vi "VirtualATE_V3.vi"() -> ()   [LabVIEW 2026]
uses:
  <vilib>/NI/Modbus Library/API/Modbus API.lvclass/Modbus API.ctl
  <vilib>/NI/Modbus Library/Transmission Data Unit/Transmission Data Unit.lvclass/Transmission Data Unit.ctl
  <vilib>/NI/Modbus Library/Transmission Data Unit/Write Unit ID.vi
  <vilib>/NI/Modbus Library/API/Read Transmission Data Unit.vi
  <vilib>/NI/Modbus Library/API/Write Transmission Data Unit.vi
  <vilib>/NI/Modbus Library/API/Master/Modbus Master.lvclass
  <vilib>/NI/Modbus Library/API/Wrapper/Create TCP Master.vi
  <vilib>/NI/Modbus Library/API/Wrapper/API Main.lvlib
panel:
  in  "Tab Control":enum32{"검사 운영", "통신 진단"}(tab)
  in  "AutoVoltage":bool=TRUE
  in  "SimVoltage_mV":i32=3300
  in  "Low_mV":i32=3000
  in  "High_mV":i32=3600
  in  "검사 결과 선택":enum16{"PASS", "FAIL", "RETEST"}(ring)
  out "ACTIVE_ID":u16
  out "ACTIVE_RESULT":u16
  out "ACTIVE_RECORD":string
  in  "Server IP":string="192.168.0.5"
  in  "Port":u16=1502
  in  "Unit ID":u8=1
  out "error out":errorcluster
  out "처리 메시지":string
  in  "LogFilePath":path
  out "ATE_STATE":u16
  out "ATE_READY":bool
  out "PLC_LIVE_OK":bool
  in  "ATE 읽기 정지":bool
  out "ATE_REQUEST":u16
  out "ATE_REQUEST_ID":u16
  out "ATE_RESULT":u16
  out "ATE_RESPONSE_ID":u16
  out "ATE_DONE":u16
  out "TEEST_RESULT_LATCH":u16
  out "SEQ_STATE":u16
  out "ALARM_CODE":u16
  out "PLC_RX_RESULT":u16
  out "PLC_RX_DONE":u16
  out "PLC_RX_RESPONSE_ID":u16
  out "PLC_ACCEPTED_ID":u16
  out "PLC_LIVE_COUNTER":u16
  out "수신 레지스터":u16[](array[numeric])
  out "마지막 Modbus 읽기 정상":bool
  out "PLC_HB_TIMEOUT":bool
  out "STATE_ELAPSED_MS":u32
  out "PLC_HB_AGE_MS":u32
  out "바깥 Tick Count(ms)":u32
  # "검사 조건"
  # "진행 중 검사"
  # "활성 요청 ID"
  # "전압 기준 자동 판정"
  # "가상 전압(mV)"
  # "하한(mV)"
  # "상한(mV)"
  # "활성 결과코드"
  # "0 없음    1 PASS    2 FAIL    3 RETEST"
  # "자동 판정 OFF 일 때 사용"
  # "캡처한 검사 레코드"
  # "Modbus 접속 설정 (실행 전)"
  # "서버 IP"
  # "포트"
  # "국번"
  # "수신 레지스터"
  # "R[1]"
  # "검사 요청"
  # "R[8]"
  # "LS 알람 코드"
  # "R[2]"
  # "검사 요청 ID"
  # "R[9]"
  # "PLC 수신 결과"
  # "R[3]"
  # "ATE 결과 워드"
  # "PLC 수신 DONE"
  # "R[10]"
  # "R[4]"
  # "ATE 응답 ID"
  # "R[11]"
  # "PLC 수신 응답 ID"
  # "R[5]"
  # "ATE 완료 워드"
  # "R[12]"
  # "PLC 수락 ID"
  # "R[6]"
  # "PLC 수락 결과"
  # "PLC 생존 카운터"
  # "R[13]"
  # "R[7]"
  # "LS 공정 상태"
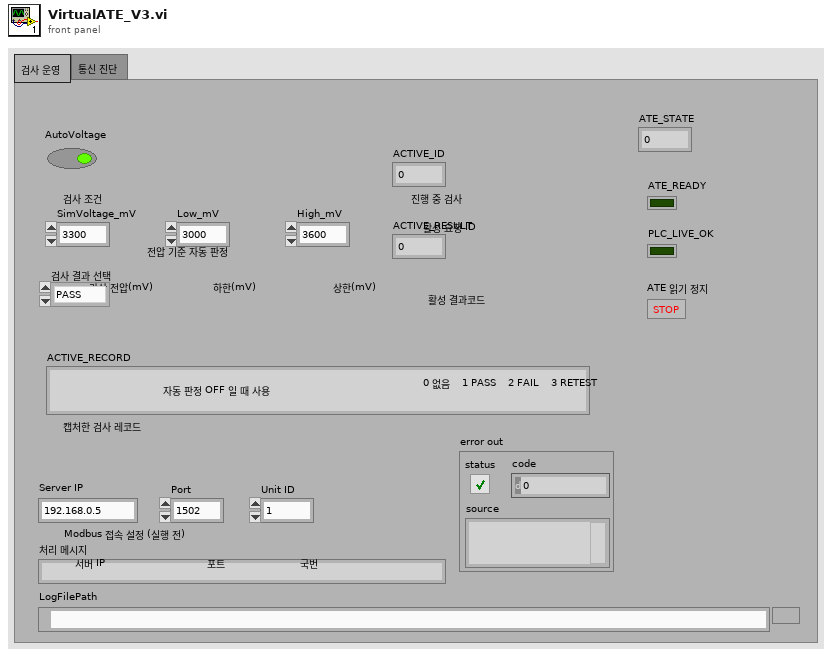
[diagram p1: front panel]
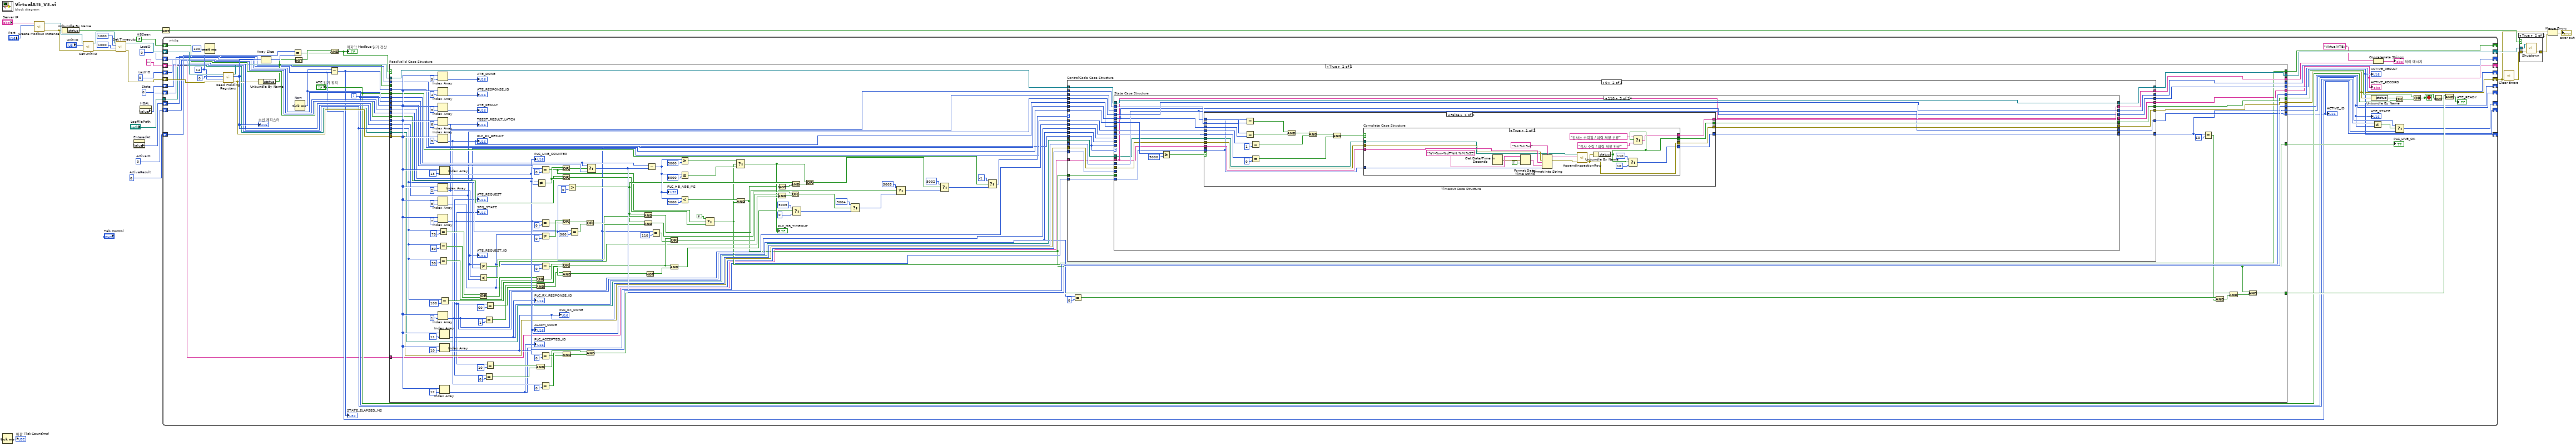
[diagram p0: block diagram]
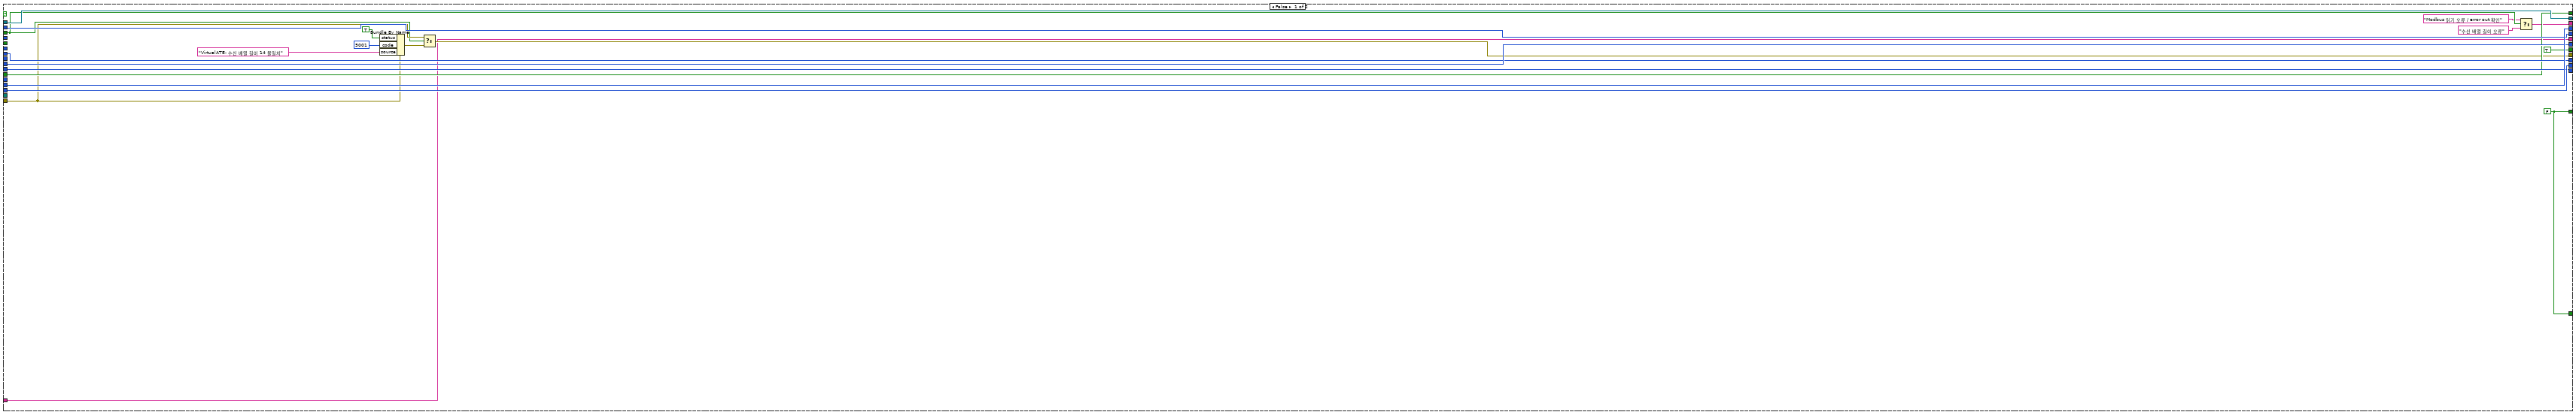
[diagram p3: hidden frame]
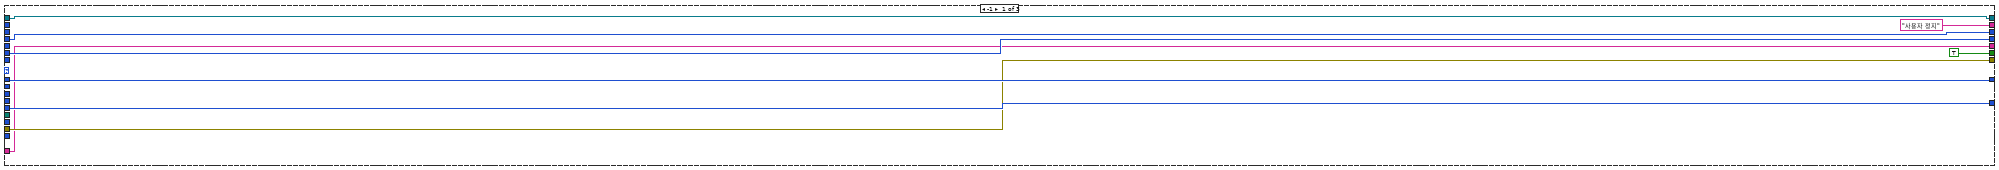
[diagram p4: hidden frame]
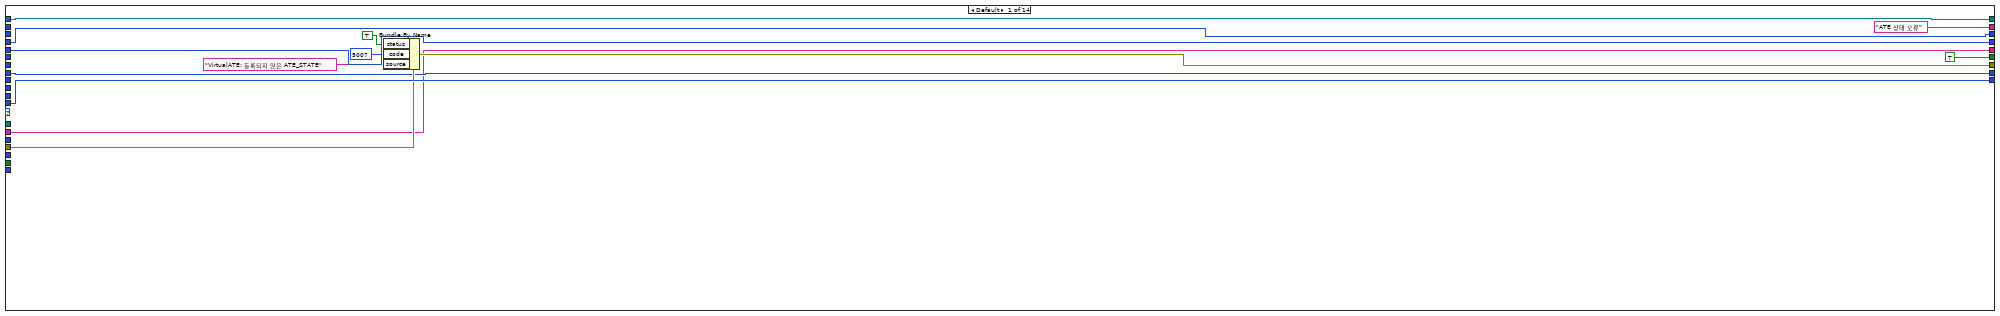
[diagram p5: hidden frame]
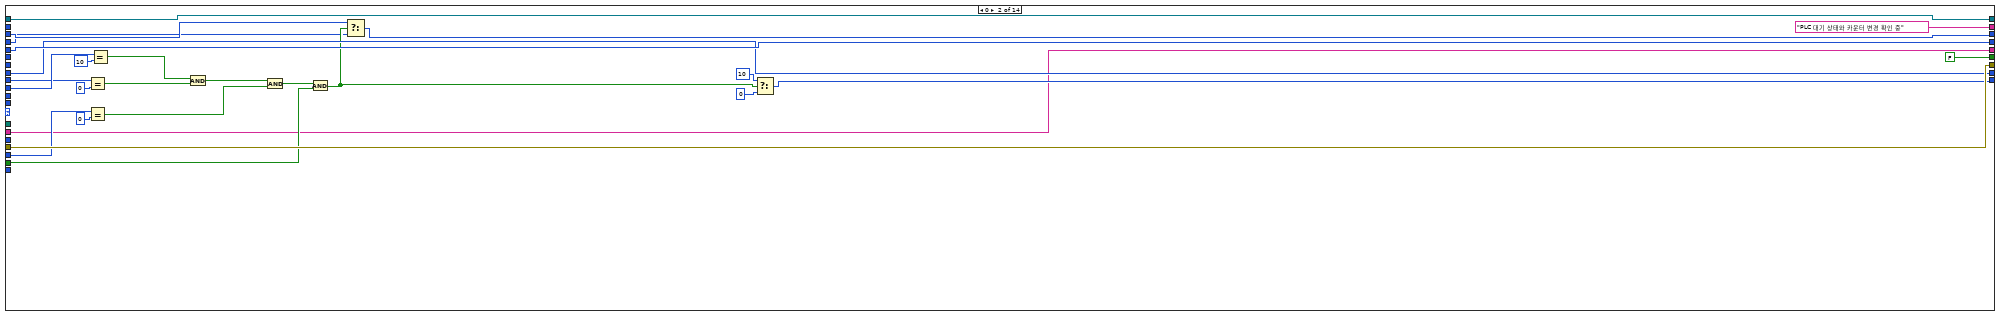
[diagram p6: hidden frame]
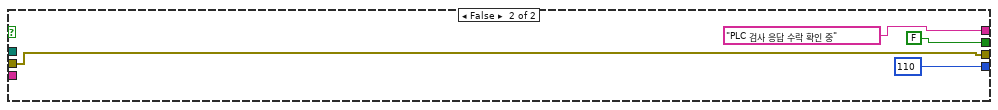
[diagram p7: hidden frame]
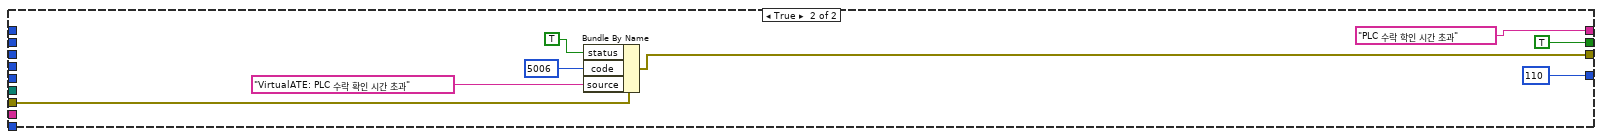
[diagram p8: hidden frame]
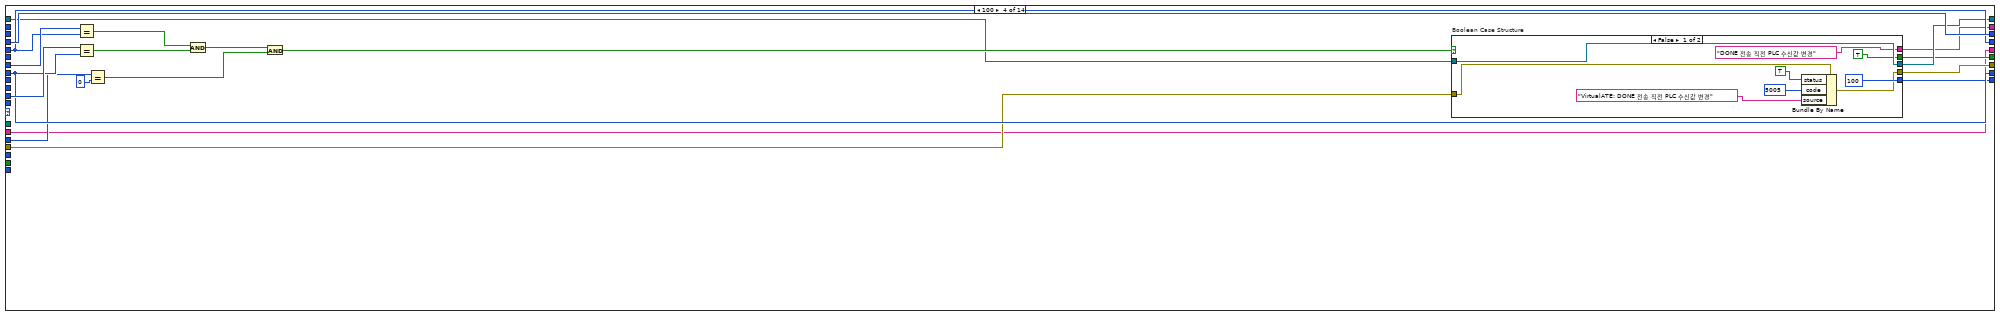
[diagram p9: hidden frame]
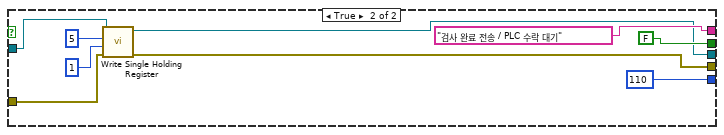
[diagram p10: hidden frame]
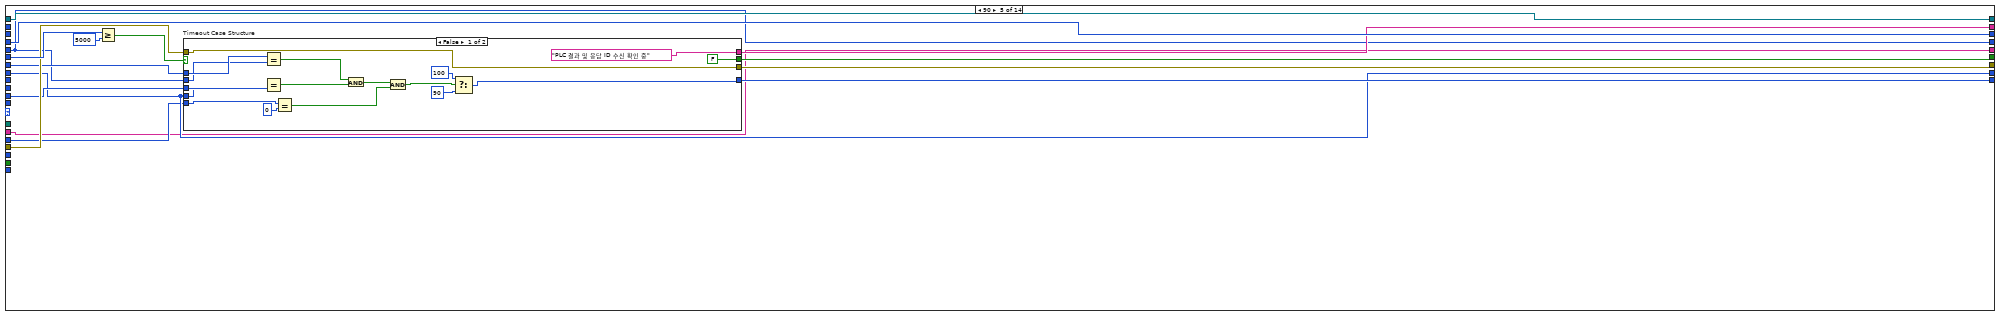
[diagram p11: hidden frame]
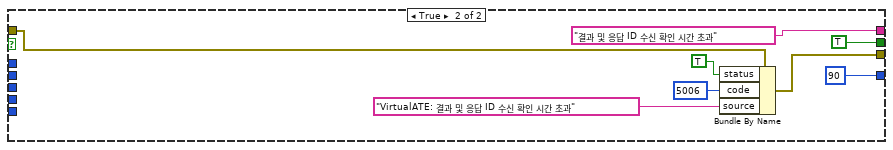
[diagram p12: hidden frame]
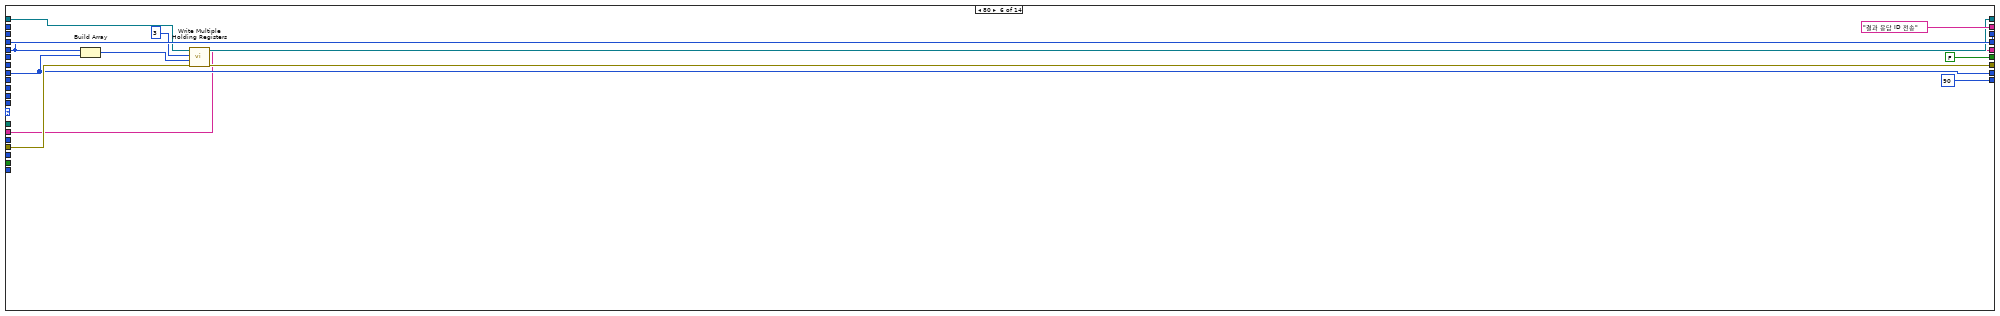
[diagram p13: hidden frame]
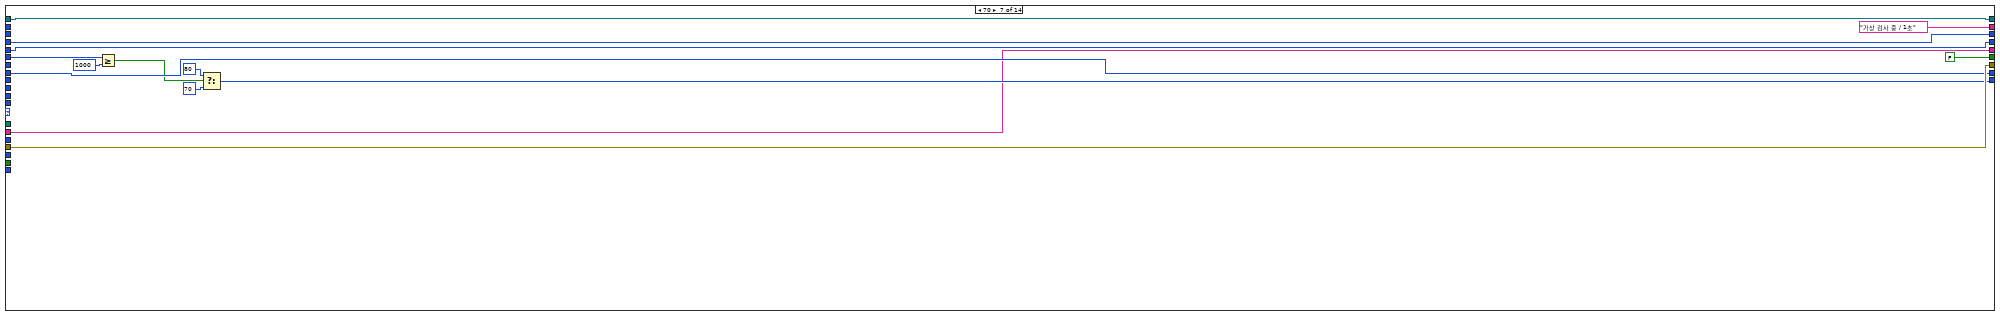
[diagram p14: hidden frame]
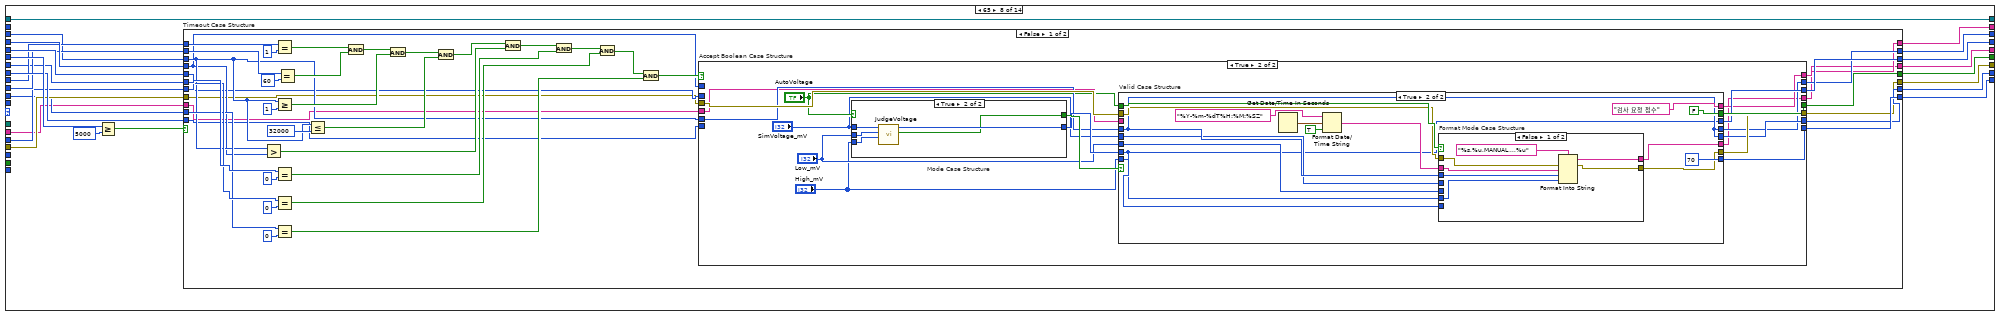
[diagram p15: hidden frame]
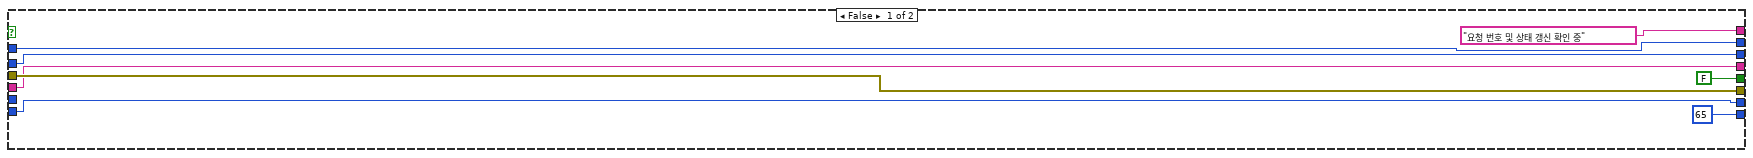
[diagram p16: hidden frame]
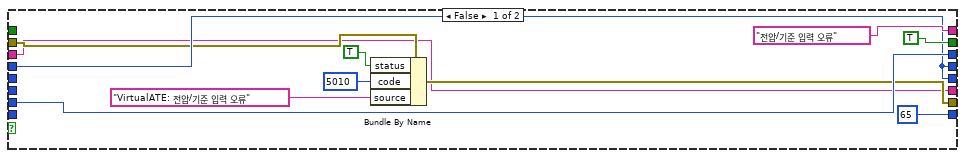
[diagram p17: hidden frame]
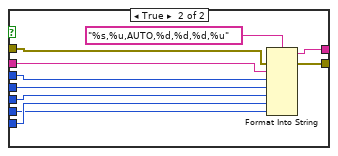
[diagram p18: hidden frame]
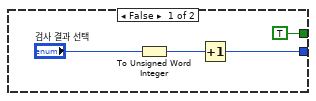
[diagram p19: hidden frame]
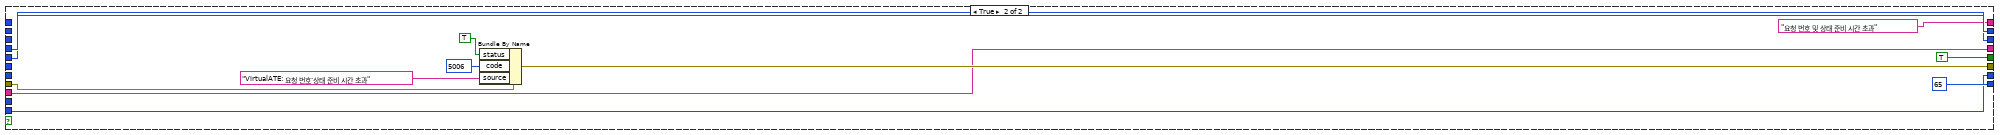
[diagram p20: hidden frame]
diagram:
  w11 = FALSE  # HBSeen
  w6 = u16 0  # LastHB
  w7 = u16 0  # ActiveResult
  w8 = u16 0  # ActiveID
  w9 = u16 0  # LastID
  w10 = u16 0  # State
  n1 = Tick Count (ms)() -> (millisecond timer value=→"바깥 Tick Count(ms)":u32)
  n2 = call-poly <vilib>:"Create Modbus Instance.vi"("port (502)"="Port", "address"="Server IP") -> ("error out"=w19:errorcluster, "TCP master instance"=w24:refnum<class "Modbus Master.lvclass">)  [unwired: 8 in]
  n3 = Unbundle By Name(w19) -> ("status"=w18:bool)
  n4 = call <vilib>:"Set Unit ID.vi"("error in"=w19, "unit ID"="Unit ID", "Modbus master in"=w24) -> ("error out"=w22:errorcluster, "Modbus master out"=w23:refnum<class "Modbus Master.lvclass">)  [unwired: 7 in]
  n5 = call <vilib>:"Set Timeouts.vi"("error in"=w22, "write operation timeout"=1000, "read operation timeout"=1000, "Modbus master in"=w23) -> ("error out"=w20:errorcluster, "Modbus master out"=w21:refnum<class "Modbus Master.lvclass">)  [unwired: 6 in]
  n6 = property on="EnteredAt" class="DigNum (strict)"() -> ("Value"=w4:u32)  [unwired: 2 in, 2 out]
  n7 = property on="HBAt" class="DigNum (strict)"() -> ("Value"=w3:u32)  [unwired: 2 in, 2 out]
  n8 = Not(x=w18) -> (.not. x?=w17:bool)
  n9 = while {
    shift-right: [w53] -> w13
    shift-left: w20 -> [w76]
    shift-right: [w64] -> w16
    shift-left: w21 -> [w77]
    shift-right: [w33] -> _
    shift-left: w10 -> [w45]
    shift-right: [w68] -> _
    shift-left: w9 -> [w69]
    shift-right: [w35] -> _
    shift-left: w8 -> [w67]
    shift-right: [w34] -> _
    shift-left: w7 -> [w66]
    shift-right: [w43] -> _
    shift-left: w3 -> [w60]
    shift-right: [w61] -> _
    shift-left: w6 -> [w62]
    shift-right: [w47] -> _
    shift-left: w4 -> [w44]
    shift-right: [w42] -> _
    shift-left: w11 -> [w59]
    shift-right: [w31] -> _
    shift-left: "" -> [w32]
    tunnel: "LogFilePath" -> [w30]
    i -> [w48]
    stop <- w50 stop-if-true
    w75 = u16 14 ("number of inputs")
    n10 = Wait (ms)(milliseconds to wait=u32 100) -> ()  [unwired: 1 out]
    n11 = call-dynamic "Read Holding Registers.vi"("error in"=w76, "number of inputs"=w75, "starting address"=u16 0, "Modbus master in"=w77) -> ("error out"=w63:errorcluster, "register values"=w71:u16[], "Modbus master out"=w65:refnum<class "Modbus Master.lvclass">)  [unwired: 5 in]
    "수신 레지스터" <- w71
    n12 = Unbundle By Name(w63) -> ("status"=w58:bool)
    n13 = Array Size(array=w71) -> (size(s)=w74:i32)
    n14 = Equal?(x=w75, y=w74) -> (x = y?=w72:bool)
    n15 = Not(x=w58) -> (.not. x?=w73:bool)
    n16 = Tick Count (ms) "Now"() -> (millisecond timer value=w41:u32)
    n17 = And(x=w73, y=w72) -> (x .and. y?=w70:bool)
    "마지막 Modbus 읽기 정상" <- w70
    n18 = Subtract(x=w41, y=w44) -> (x-y=w39:u32)
    "STATE_ELAPSED_MS" <- w39
    n19 = case "ReadValid Case Structure" shown="True" w70 {
      tunnel: w71 -> [_ w229]
      tunnel: w45 -> [w100 w136]
      tunnel: [w100 w130] -> w33
      tunnel: w69 -> [w99 w148]
      tunnel: [w99 w147] -> w68
      tunnel: w67 -> [w98 w146]
      tunnel: [w98 w145] -> w35
      tunnel: w66 -> [w97 w144]
      tunnel: [w97 w143] -> w34
      tunnel: w65 -> [w96 w142]
      tunnel: [w96 w141] -> w64
      tunnel: w63 -> [w88 w140]
      tunnel: [w82 w139] -> w53
      tunnel: w62 -> [w95 w221]
      tunnel: [w95 w218] -> w61
      tunnel: w60 -> [w94 w216]
      tunnel: [w94 w217] -> w43
      tunnel: w59 -> [w93 w219]
      tunnel: [w93 w111] -> w42
      tunnel: w58 -> [w86 _]
      tunnel: [TRUE w137] -> w56
      tunnel: [w83 w138] -> w37
      tunnel: [w81 w117] -> w54
      tunnel: [w81 w104] -> w49
      tunnel: w48 -> [_ w223]
      tunnel: w41 -> [_ w210]
      tunnel: "ATE 읽기 정지" -> [_ w150]
      tunnel: w39 -> [_ w116]
      tunnel: w32 -> [w80 w103]
      tunnel: [w80 w102] -> w31
      tunnel: w30 -> [_ w101]
      frame False {
        w81 = FALSE
        n20 = Bundle By Name(cluster=w88, "status"=TRUE, "code"=5001, "source"="VirtualATE: 수신 배열 길이 14 불일치") -> (w89:errorcluster)
        n21 = Select(t=w88, s=w86, f=w89) -> (s? t:f=w82:errorcluster)
        n22 = Select(t="Modbus 읽기 오류 / error out 확인", s=w86, f="수신 배열 길이 오류") -> (s? t:f=w83:string)
      }
      frame True {
        n23 = Index Array(array=w229, index=5) -> (element=→"ATE_DONE":u16)
        n24 = Index Array(array=w229, index=4) -> (element=→"ATE_RESPONSE_ID":u16)
        n25 = Index Array(array=w229, index=3) -> (element=→"ATE_RESULT":u16)
        n26 = Index Array(array=w229, index=6) -> (element=w105:u16)
        "TEEST_RESULT_LATCH" <- w105
        n27 = Index Array(array=w229, index=9) -> (element=w114:u16)
        "PLC_RX_RESULT" <- w114
        n28 = Index Array(array=w229, index=2) -> (element=w107:u16)
        "ATE_REQUEST_ID" <- w107
        n29 = Index Array(array=w229, index=8) -> (element=w108:u16)
        "ALARM_CODE" <- w108
        n30 = Index Array(array=w229, index=7) -> (element=w109:u16)
        "SEQ_STATE" <- w109
        n31 = Index Array(array=w229, index=1) -> (element=w112:u16)
        "ATE_REQUEST" <- w112
        n32 = Equal?(x=w136, y=u16 70) -> (x = y?=w199:bool)
        n33 = Equal?(x=w136, y=u16 80) -> (x = y?=w198:bool)
        n34 = Equal?(x=w136, y=u16 90) -> (x = y?=w197:bool)
        n35 = Index Array(array=w229, index=13) -> (element=w218:u16)
        "PLC_LIVE_COUNTER" <- w218
        n36 = Index Array(array=w229, index=11) -> (element=w113:u16)
        "PLC_RX_RESPONSE_ID" <- w113
        n37 = Index Array(array=w229, index=10) -> (element=w115:u16)
        "PLC_RX_DONE" <- w115
        n38 = Index Array(array=w229, index=12) -> (element=w106:u16)
        "PLC_ACCEPTED_ID" <- w106
        n39 = Equal?(x=w136, y=u16 100) -> (x = y?=w195:bool)
        n40 = Not Equal?(x=w107, y=w146) -> (x != y?=w179:bool)
        n41 = Less?(x=w107, y=w148) -> (x < y?=w181:bool)
        n42 = Or(x=w199, y=w198) -> (x .or. y?=w196:bool)
        n43 = Equal?(x=w112, y=u16 1) -> (x = y?=w188:bool)
        n44 = Equal?(x=w112, y=u16 0) -> (x = y?=w127:bool)
        n45 = Equal?(x=w109, y=u16 60) -> (x = y?=w187:bool)
        n46 = Equal?(x=w109, y=u16 10) -> (x = y?=w128:bool)
        n47 = Or(x=w196, y=w197) -> (x .or. y?=w194:bool)
        n48 = And(x=w188, y=w187) -> (x .and. y?=w185:bool)
        n49 = And(x=w128, y=w127) -> (x .and. y?=w122:bool)
        n50 = Not Equal?(x=w218, y=w221) -> (x != y?=w220:bool)
        n51 = Equal?(x=w223, y=0) -> (x = y?=w110:bool)
        n52 = Equal?(x=w109, y=u16 0) -> (x = y?=w172:bool)
        n53 = Not Equal?(x=w108, y=u16 0) -> (x != y?=w173:bool)
        n54 = Equal?(x=w108, y=u16 0) -> (x = y?=w186:bool)
        n55 = Equal?(x=w115, y=u16 0) -> (x = y?=w125:bool)
        n56 = Equal?(x=w114, y=u16 0) -> (x = y?=w126:bool)
        n57 = Or(x=w220, y=w110) -> (x .or. y?=w214:bool)
        n58 = Or(x=w219, y=w220) -> (x .or. y?=w215:bool)
        n59 = Or(x=w173, y=w172) -> (x .or. y?=w171:bool)
        n60 = Or(x=w194, y=w195) -> (x .or. y?=w182:bool)
        n61 = And(x=w185, y=w186) -> (x .and. y?=w184:bool)
        n62 = And(x=w126, y=w125) -> (x .and. y?=w121:bool)
        n63 = Greater?(x=w136, y=u16 0) -> (0:w168:bool)
        n64 = Equal?(x=w109, y=u16 900) -> (x = y?=w170:bool)
        n65 = Or(x=w171, y=w170) -> (x .or. y?=w169:bool)
        n66 = And(x=w122, y=w121) -> (x .and. y?=w119:bool)
        n67 = Select(t=w210, s=w214, f=w216) -> (s? t:f=w217:u32)
        n68 = And(x=w168, y=w169) -> (x .and. y?=w160:bool)
        n69 = And(x=w168, y=w181) -> (x .and. y?=w178:bool)
        n70 = Not(x=w184) -> (.not. x?=w183:bool)
        n71 = Subtract(x=w210, y=w217) -> (x-y=w209:u32)
        "PLC_HB_AGE_MS" <- w209
        n72 = Equal?(x=w136, y=u16 110) -> (x = y?=w192:bool)
        n73 = Or(x=w182, y=w192) -> (x .or. y?=w180:bool)
        n74 = And(x=w182, y=w183) -> (x .and. y?=w164:bool)
        n75 = Greater Or Equal?(x=w209, y=u32 3000) -> (x >= y?=w206:bool)
        n76 = Greater Or Equal?(x=w209, y=u32 5000) -> (x >= y?=w205:bool)
        n77 = Less?(x=w209, y=u32 3000) -> (x < y?=w212:bool)
        n78 = Select(t=FALSE, s=w110, f=w215) -> (s? t:f=w111:bool)
        n79 = Select(t=w206, s=w111, f=w205) -> (s? t:f=w165:bool)
        "PLC_HB_TIMEOUT" <- w165
        n80 = And(x=w212, y=w111) -> (x .and. y?=w104:bool)
        n81 = Not(x=w104) -> (.not. x?=w167:bool)
        n82 = And(x=w180, y=w179) -> (x .and. y?=w177:bool)
        n83 = Or(x=w178, y=w177) -> (x .or. y?=w161:bool)
        n84 = And(x=w168, y=w167) -> (x .and. y?=w166:bool)
        n85 = Select(t=5005, s=w164, f=0) -> (s? t:f=w157:i32)
        n86 = Or(x=w165, y=w166) -> (x .or. y?=w159:bool)
        n87 = Select(t=5004, s=w161, f=w157) -> (s? t:f=w156:i32)
        n88 = Select(t=5003, s=w160, f=w156) -> (s? t:f=w154:i32)
        n89 = Select(t=5002, s=w159, f=w154) -> (s? t:f=w152:i32)
        n90 = Select(t=-1, s=w150, f=w152) -> (s? t:f=w149:i32)
        n91 = case "ControlCode Case Structure" shown="0" w149 {
          selector: w149 -> [_ _ w817]
          tunnel: w136 -> [w249 w260 w825]
          tunnel: [w249 w271 w825] -> w130
          tunnel: w148 -> [w248 w277 w824]
          tunnel: [w248 w268 w824] -> w147
          tunnel: w146 -> [w247 w276 w823]
          tunnel: [w247 w267 w823] -> w145
          tunnel: [w246 w273 w822] -> w143
          tunnel: w144 -> [w246 w275 w822]
          tunnel: [w245 w272 w821] -> w141
          tunnel: w142 -> [w245 w274 w821]
          tunnel: [w244 w270 w820] -> w139
          tunnel: w140 -> [w244 w269 w819]
          tunnel: ["사용자 정지" w265 w799] -> w138
          tunnel: [TRUE w266 TRUE] -> w137
          tunnel: w116 -> [_ w264 _]
          tunnel: w115 -> [_ w263 _]
          tunnel: w114 -> [_ w262 _]
          tunnel: w113 -> [_ w261 _]
          tunnel: w112 -> [_ w257 _]
          tunnel: w109 -> [_ w259 _]
          tunnel: w108 -> [_ w258 _]
          tunnel: w107 -> [_ w256 _]
          tunnel: w106 -> [_ w255 _]
          tunnel: w105 -> [_ w254 _]
          tunnel: w104 -> [_ w253 _]
          tunnel: w103 -> [w241 w252 w798]
          tunnel: [w241 w251 w798] -> w102
          tunnel: w101 -> [_ w250 _]
          frame -1 {
          }
          frame 0 {
            n92 = case "State Case Structure" shown="110" w260 {
              tunnel: w277 -> [w279 w293 w333 w407 w440 w478 w490 w511 w658 w692 w710 w751 w765 w795]
              tunnel: w276 -> [w280 w313 w320 w403 w428 w468 w489 w507 w657 w691 w709 w750 w764 w794]
              tunnel: w275 -> [w289 w316 w319 w405 w430 w469 w493 w505 w661 w695 w712 w753 w767 w797]
              tunnel: w274 -> [w288 w315 w334 w393 w441 w472 w492 w516 w660 w694 w711 w747 w766 w791]
              tunnel: [w289 w316 w319 w405 w430 w469 w493 w504 w661 w695 w712 w753 w767 w797] -> w273
              tunnel: [w288 w315 w334 w392 w441 w470 w492 w516 w660 w694 w711 w745 w766 w790] -> w272
              tunnel: [w290 w295 w329 w390 w434 u16 90 w484 w512 w649 w665 w703 u16 40 w758 u16 20] -> w271
              tunnel: [w283 w314 w325 w394 w435 w471 w491 w502 w659 w693 w701 w744 w757 w789] -> w270
              tunnel: w269 -> [w287 w314 w326 w395 w436 w473 w491 w503 w659 w693 w702 w746 w756 w788]
              tunnel: [w279 w292 w333 w407 w440 w478 w490 w510 w658 w692 w710 w751 w765 w795] -> w268
              tunnel: [w280 w313 w320 w403 w428 w468 w489 w506 w657 w691 w709 w750 w764 w794] -> w267
              tunnel: [TRUE FALSE w328 w391 w433 FALSE FALSE w509 FALSE FALSE w705 FALSE w759 FALSE] -> w266
              tunnel: ["ATE 상태 오류" "PLC 대기 상태와 카운터 변경 확인 중" w327 w389 w432 "결과 응답 ID 전송" "가상 검사 중 / 1초" w508 "새 검사 요청 대기" "분류 및 배출 완료 후 PLC 대기 복귀 확인" w704 "결과 및 응답 ID 초기화 전송" w760 "DONE=0 전송 / PLC 반영 대기"] -> w265
              tunnel: w260 -> [w290 _ _ _ _ _ _ _ _ _ _ _ _ _]
              tunnel: w264 -> [_ _ w332 _ w439 _ w482 w514 _ _ w707 _ w762 _]
              tunnel: w263 -> [_ _ w322 w402 w427 _ _ w497 _ w684 w699 _ w755 _]
              tunnel: w262 -> [_ _ _ w406 w431 _ _ w498 _ w685 w700 _ _ _]
              tunnel: w261 -> [_ _ _ w404 w429 _ _ w496 _ w683 w698 _ _ _]
              tunnel: w257 -> [_ w308 w321 _ _ _ _ w501 w654 w687 w697 _ _ _]
              tunnel: w259 -> [_ w310 _ _ _ _ _ w500 _ w688 _ _ _ _]
              tunnel: w258 -> [_ w307 _ _ _ _ _ _ _ w686 _ _ _ _]
              tunnel: w256 -> [_ w294 _ _ _ _ _ w499 _ _ _ _ _ _]
              tunnel: w255 -> [_ _ w324 _ _ _ _ _ _ _ _ _ _ _]
              tunnel: w254 -> [_ _ w323 _ _ _ _ _ _ _ _ _ _ _]
              tunnel: w253 -> [_ w299 _ _ _ _ _ _ _ _ _ _ _ _]
              tunnel: w252 -> [w278 w291 w318 w388 w426 w467 w480 w495 w648 w662 w696 w739 w754 w785]
              tunnel: [w278 w291 w318 w388 w426 w467 w480 w494 w648 w662 w696 w739 w754 w785] -> w251
              tunnel: w250 -> [_ _ w317 _ _ _ _ _ _ _ _ _ _ _]
              frame Default {
                n93 = Bundle By Name(cluster=w287, "status"=TRUE, "code"=5007, "source"="VirtualATE: 등록되지 않은 ATE_STATE") -> (w283:errorcluster)
              }
              frame 0 {
                n94 = Equal?(x=w308, y=u16 0) -> (x = y?=w303:bool)
                n95 = Equal?(x=w307, y=u16 0) -> (x = y?=w302:bool)
                n96 = Equal?(x=w310, y=u16 10) -> (x = y?=w304:bool)
                n97 = And(x=w304, y=w303) -> (x .and. y?=w301:bool)
                n98 = And(x=w301, y=w302) -> (x .and. y?=w300:bool)
                n99 = And(x=w300, y=w299) -> (x .and. y?=w298:bool)
                n100 = Select(t=w294, s=w298, f=w293) -> (s? t:f=w292:u16)
                n101 = Select(t=u16 10, s=w298, f=u16 0) -> (s? t:f=w295:u16)
              }
              frame 110 {
                n102 = Greater Or Equal?(x=w332, y=u32 5000) -> (x >= y?=w330:bool)
                n103 = case "Timeout Case Structure" shown="False" w330 {
                  tunnel: [w342 u16 110] -> w329
                  tunnel: [w341 TRUE] -> w328
                  tunnel: [w340 "PLC 수락 학인 시간 초과"] -> w327
                  tunnel: w326 -> [w339 w384]
                  tunnel: [w338 w380] -> w325
                  tunnel: w324 -> [w336 _]
                  tunnel: w323 -> [w356 _]
                  tunnel: w322 -> [w355 _]
                  tunnel: w321 -> [w354 _]
                  tunnel: w320 -> [w353 _]
                  tunnel: w319 -> [w352 _]
                  tunnel: w318 -> [w337 _]
                  tunnel: w317 -> [w335 _]
                  frame False {
                    n104 = Equal?(x=w336, y=w353) -> (x = y?=w349:bool)
                    n105 = Equal?(x=w356, y=w352) -> (x = y?=w348:bool)
                    n106 = Equal?(x=w355, y=u16 1) -> (x = y?=w347:bool)
                    n107 = Equal?(x=w354, y=u16 0) -> (x = y?=w346:bool)
                    n108 = And(x=w349, y=w348) -> (x .and. y?=w345:bool)
                    n109 = And(x=w345, y=w347) -> (x .and. y?=w344:bool)
                    n110 = And(x=w344, y=w346) -> (x .and. y?=w343:bool)
                    n111 = case "Complete Case Structure" shown="True" w343 {
                      tunnel: [w360 u16 110] -> w342
                      tunnel: [w363 FALSE] -> w341
                      tunnel: [w357 "PLC 검사 응답 수락 확인 중"] -> w340
                      tunnel: w339 -> [w368 w376]
                      tunnel: [w364 w376] -> w338
                      tunnel: w337 -> [w372 _]
                      tunnel: w336 -> [w369 _]
                      tunnel: w335 -> [w367 _]
                      frame True {
                        n112 = Get Date/Time In Seconds() -> (seconds since 1Jan1904=w370:timestamp)
                        n113 = Format Date/Time String(time format string (%c)="%Y-%m-%dT%H:%M:%SZ", seconds (now)=w370, UTC format=TRUE) -> (date/time string=w371:string)
                        n114 = Format Into String(format string="%s,%s,%u", error in=w368, w372, w371, w369) -> (resulting string=w366:string, error out=w365:errorcluster)  [unwired: 1 in]
                        n115 = call "AppendInspectionRow.vi"("error in (no error)"=w365, "Row"=w366, "FilePath"=w367) -> ("error out"=w364:errorcluster)  [unwired: 6 in]
                        n116 = Unbundle By Name(w364) -> ("status"=w363:bool)
                        n117 = Select(t=u16 110, s=w363, f=u16 10) -> (s? t:f=w360:u16)
                        n118 = Select(t="검사는 수락됨 / 이력 저장 오류", s=w363, f="검사 수락 / 이력 저장 완료") -> (s? t:f=w357:string)
                      }
                      frame False {
                      }
                    }
                  }
                  frame True {
                    n119 = Bundle By Name(cluster=w384, "status"=TRUE, "code"=5006, "source"="VirtualATE: PLC 수락 확인 시간 초과") -> (w380:errorcluster)
                  }
                }
              }
              frame 100 {
                n120 = Equal?(x=w406, y=w405) -> (x = y?=w400:bool)
                n121 = Equal?(x=w404, y=w403) -> (x = y?=w399:bool)
                n122 = Equal?(x=w402, y=u16 0) -> (x = y?=w398:bool)
                n123 = And(x=w400, y=w399) -> (x .and. y?=w397:bool)
                n124 = And(x=w397, y=w398) -> (x .and. y?=w396:bool)
                n125 = case "Boolean Case Structure" shown="False" w396 {
                  tunnel: w395 -> [w412 w420]
                  tunnel: [w408 w419] -> w394
                  tunnel: w393 -> [w415 w422]
                  tunnel: [w415 w421] -> w392
                  tunnel: [TRUE FALSE] -> w391
                  tunnel: [u16 100 u16 110] -> w390
                  tunnel: ["DONE 전송 직전 PLC 수신값 변경" "검사 완료 전송 / PLC 수락 대기"] -> w389
                  frame False {
                    n126 = Bundle By Name(cluster=w412, "status"=TRUE, "code"=5005, "source"="VirtualATE: DONE 전송 직전 PLC 수신값 변경") -> (w408:errorcluster)
                  }
                  frame True {
                    n127 = call-dynamic "Write Single Holding Register.vi"("error in"=w420, "register to write"=u16 1, "address"=u16 5, "Modbus master in"=w422) -> ("error out"=w419:errorcluster, "Modbus master out"=w421:refnum<class "Modbus Master.lvclass">)  [unwired: 6 in]
                  }
                }
              }
              frame 90 {
                n128 = Greater Or Equal?(x=w439, y=u32 5000) -> (x >= y?=w437:bool)
                n129 = case "Timeout Case Structure" shown="False" w437 {
                  tunnel: w436 -> [w458 w466]
                  tunnel: [w458 w462] -> w435
                  tunnel: [w442 u16 90] -> w434
                  tunnel: [FALSE TRUE] -> w433
                  tunnel: ["PLC 결과 및 응답 ID 수신 확인 중" "결과 및 응답 ID 수신 확인 시간 초과"] -> w432
                  tunnel: w431 -> [w455 _]
                  tunnel: w430 -> [w454 _]
                  tunnel: w429 -> [w453 _]
                  tunnel: w428 -> [w452 _]
                  tunnel: w427 -> [w451 _]
                  frame False {
                    n130 = Equal?(x=w455, y=w454) -> (x = y?=w449:bool)
                    n131 = Equal?(x=w453, y=w452) -> (x = y?=w448:bool)
                    n132 = Equal?(x=w451, y=u16 0) -> (x = y?=w447:bool)
                    n133 = And(x=w449, y=w448) -> (x .and. y?=w446:bool)
                    n134 = And(x=w446, y=w447) -> (x .and. y?=w445:bool)
                    n135 = Select(t=u16 100, s=w445, f=u16 90) -> (s? t:f=w442:u16)
                  }
                  frame True {
                    n136 = Bundle By Name(cluster=w466, "status"=TRUE, "code"=5006, "source"="VirtualATE: 결과 및 응답 ID 수신 확인 시간 초과") -> (w462:errorcluster)
                  }
                }
              }
              frame 80 {
                n137 = Build Array(w469, w468) -> (w474:u16[])
                n138 = call-dynamic "Write Multiple Holding Registers.vi"("error in"=w473, "registers to write"=w474, "starting address"=u16 3, "Modbus master in"=w472) -> ("error out"=w471:errorcluster, "Modbus master out"=w470:refnum<class "Modbus Master.lvclass">)  [unwired: 6 in]
              }
              frame 70 {
                n139 = Greater Or Equal?(x=w482, y=u32 1000) -> (x >= y?=w483:bool)
                n140 = Select(t=u16 80, s=w483, f=u16 70) -> (s? t:f=w484:u16)
              }
              frame 65 {
                n141 = Greater Or Equal?(x=w514, y=u32 5000) -> (x >= y?=w513:bool)
                n142 = case "Timeout Case Structure" shown="False" w513 {
                  tunnel: [w530 u16 65] -> w512
                  tunnel: w511 -> [w524 w646]
                  tunnel: [w527 w646] -> w510
                  tunnel: [w520 TRUE] -> w509
                  tunnel: [w525 "요청 번호 및 상태 준비 시간 초과"] -> w508
                  tunnel: w507 -> [w523 w643]
                  tunnel: [w526 w643] -> w506
                  tunnel: w505 -> [w522 w642]
                  tunnel: [w528 w642] -> w504
                  tunnel: w503 -> [w519 w641]
                  tunnel: [w521 w637] -> w502
                  tunnel: w501 -> [w557 _]
                  tunnel: w500 -> [w555 _]
                  tunnel: w499 -> [w529 _]
                  tunnel: w498 -> [w543 _]
                  tunnel: w497 -> [w537 _]
                  tunnel: w496 -> [w534 _]
                  tunnel: w495 -> [w518 w636]
                  tunnel: [w517 w636] -> w494
                  frame False {
                    n143 = Greater?(x=w529, y=w524) -> (0:w544:bool)
                    n144 = Equal?(x=w557, y=u16 1) -> (x = y?=w553:bool)
                    n145 = Greater Or Equal?(x=w529, y=u16 1) -> (x >= y?=w549:bool)
                    n146 = Equal?(x=w543, y=u16 0) -> (x = y?=w538:bool)
                    n147 = Equal?(x=w537, y=u16 0) -> (x = y?=w535:bool)
                    n148 = Equal?(x=w534, y=u16 0) -> (x = y?=w532:bool)
                    n149 = Equal?(x=w555, y=u16 60) -> (x = y?=w552:bool)
                    n150 = Less Or Equal?(x=w529, y=u16 32000) -> (x <= y?=w546:bool)
                    n151 = And(x=w553, y=w552) -> (x .and. y?=w550:bool)
                    n152 = And(x=w550, y=w549) -> (x .and. y?=w547:bool)
                    n153 = And(x=w547, y=w546) -> (x .and. y?=w545:bool)
                    n154 = And(x=w545, y=w544) -> (x .and. y?=w541:bool)
                    n155 = And(x=w541, y=w538) -> (x .and. y?=w540:bool)
                    n156 = And(x=w540, y=w535) -> (x .and. y?=w539:bool)
                    n157 = And(x=w539, y=w532) -> (x .and. y?=w531:bool)
                    n158 = case "Accept Boolean Case Structure" shown="True" w531 {
                      tunnel: [u16 65 w581] -> w530
                      tunnel: w529 -> [_ w574]
                      tunnel: [w562 w578] -> w528
                      tunnel: [w564 w572] -> w527
                      tunnel: [w563 w573] -> w526
                      tunnel: ["요청 번호 및 상태 갱신 확인 중" w577] -> w525
                      tunnel: w524 -> [w564 _]
                      tunnel: w523 -> [w563 _]
                      tunnel: w522 -> [w562 _]
                      tunnel: [w559 w575] -> w521
                      tunnel: [FALSE w580] -> w520
                      tunnel: w519 -> [w559 w576]
                      tunnel: w518 -> [w558 w571]
                      tunnel: [w558 w570] -> w517
                      frame False {
                      }
                      frame True {
                        n159 = case "Mode Case Structure" shown="True" "AutoVoltage" {
                          tunnel: [w627 w635] -> w579
                          tunnel: [TRUE ("InputValid") w634] -> w582
                          tunnel: "SimVoltage_mV" -> [_ w633]
                          tunnel: "Low_mV" -> [_ w632]
                          tunnel: "High_mV" -> [_ w631]
                          frame False {
                            n160 = To Unsigned Word Integer(number="검사 결과 선택") -> (unsigned 16bit integer=w629:u16)
                            n161 = Increment(x=w629) -> (x+1=w627:u16)
                          }
                          frame True {
                            n162 = call "JudgeVoltage.vi"("High_mV"=w631, "Low_mV"=w632, "Voltage_mV"=w633) -> ("InputValid"=w634:bool, "Result"=w635:u16)  [unwired: 7 in]
                          }
                        }
                        n163 = case "Valid Case Structure" shown="True" w582 {
                          tunnel: [u16 65 u16 70] -> w581
                          tunnel: [TRUE FALSE] -> w580
                          tunnel: w579 -> [w590 w595]
                          tunnel: [w590 w595] -> w578
                          tunnel: ["전압/기준 입력 오류" "검사 요청 접수"] -> w577
                          tunnel: w576 -> [w588 w602]
                          tunnel: [w584 w601] -> w575
                          tunnel: w574 -> [w589 w599]
                          tunnel: [w589 w599] -> w573
                          tunnel: [w589 w599] -> w572
                          tunnel: w571 -> [w583 _]
                          tunnel: [w583 w594] -> w570
                          tunnel: "AutoVoltage" -> [_ w603]
                          tunnel: "SimVoltage_mV" -> [_ w598]
                          tunnel: "Low_mV" -> [_ w597]
                          tunnel: "High_mV" -> [_ w596]
                          frame False {
                            n164 = Bundle By Name(cluster=w588, "status"=TRUE, "code"=5010, "source"="VirtualATE: 전압/기준 입력 오류") -> (w584:errorcluster)
                          }
                          frame True {
                            n165 = Get Date/Time In Seconds() -> (seconds since 1Jan1904=w606:timestamp)
                            n166 = Format Date/Time String(time format string (%c)="%Y-%m-%dT%H:%M:%SZ", seconds (now)=w606, UTC format=TRUE) -> (date/time string=w600:string)
                            n167 = case "Format Mode Case Structure" shown="False" w603 {
                              tunnel: [w616 w626] -> w594
                              tunnel: w602 -> [w615 w625]
                              tunnel: [w614 w624] -> w601
                              tunnel: w600 -> [w612 w622]
                              tunnel: w599 -> [w611 w621]
                              tunnel: w598 -> [_ w620]
                              tunnel: w597 -> [_ w619]
                              tunnel: w596 -> [_ w618]
                              tunnel: w595 -> [w610 w617]
                              frame False {
                                n168 = Format Into String(format string="%s,%u,MANUAL,,,,%u", error in=w615, w612, w611, w610) -> (resulting string=w616:string, error out=w614:errorcluster)  [unwired: 1 in]
                              }
                              frame True {
                                n169 = Format Into String(format string="%s,%u,AUTO,%d,%d,%d,%u", error in=w625, w622, w621, w620, w619, w618, w617) -> (resulting string=w626:string, error out=w624:errorcluster)  [unwired: 1 in]
                              }
                            }
                          }
                        }
                      }
                    }
                  }
                  frame True {
                    n170 = Bundle By Name(cluster=w641, "status"=TRUE, "code"=5006, "source"="VirtualATE: 요청 번호·상태 준비 시간 초과") -> (w637:errorcluster)
                  }
                }
              }
              frame 60 {
                n171 = Equal?(x=w654, y=u16 1) -> (x = y?=w652:bool)
                n172 = Select(t=u16 65, s=w652, f=u16 60) -> (s? t:f=w649:u16)
              }
              frame 50 {
                n173 = Equal?(x=w687, y=u16 0) -> (x = y?=w675:bool)
                n174 = Equal?(x=w686, y=u16 0) -> (x = y?=w674:bool)
                n175 = Equal?(x=w685, y=u16 0) -> (x = y?=w672:bool)
                n176 = Equal?(x=w684, y=u16 0) -> (x = y?=w670:bool)
                n177 = Equal?(x=w683, y=u16 0) -> (x = y?=w668:bool)
                n178 = Equal?(x=w688, y=u16 10) -> (x = y?=w676:bool)
                n179 = And(x=w676, y=w675) -> (x .and. y?=w673:bool)
                n180 = And(x=w673, y=w674) -> (x .and. y?=w671:bool)
                n181 = And(x=w671, y=w672) -> (x .and. y?=w669:bool)
                n182 = And(x=w669, y=w670) -> (x .and. y?=w667:bool)
                n183 = And(x=w667, y=w668) -> (x .and. y?=w666:bool)
                n184 = Select(t=u16 60, s=w666, f=u16 50) -> (s? t:f=w665:u16)
              }
              frame 40 {
                n185 = Greater Or Equal?(x=w707, y=u32 5000) -> (x >= y?=w706:bool)
                n186 = case "Timeout Case Structure" shown="False" w706 {
                  tunnel: [FALSE TRUE] -> w705
                  tunnel: ["PLC 응답 초기화 확인 중" "응답 초기화 확인 시간 초과"] -> w704
                  tunnel: [w725 u16 40] -> w703
                  tunnel: w702 -> [w730 w735]
                  tunnel: [w730 w731] -> w701
                  tunnel: w700 -> [w723 _]
                  tunnel: w699 -> [w722 _]
                  tunnel: w698 -> [w721 _]
                  tunnel: w697 -> [w720 _]
                  frame False {
                    w724 = u16 0 ("y")
                    n187 = Equal?(x=w723, y=w724) -> (x = y?=w719:bool)
                    n188 = Equal?(x=w722, y=w724) -> (x = y?=w718:bool)
                    n189 = Equal?(x=w721, y=w724) -> (x = y?=w717:bool)
                    n190 = Equal?(x=w720, y=w724) -> (x = y?=w716:bool)
                    n191 = And(x=w719, y=w718) -> (x .and. y?=w715:bool)
                    n192 = And(x=w717, y=w716) -> (x .and. y?=w714:bool)
                    n193 = And(x=w715, y=w714) -> (x .and. y?=w713:bool)
                    n194 = Select(t=u16 50, s=w713, f=u16 40) -> (s? t:f=w725:u16)
                  }
                  frame True {
                    n195 = Bundle By Name(cluster=w735, "status"=TRUE, "code"=5006, "source"="VirtualATE: 응답 초기화 확인 시간 초과") -> (w731:errorcluster)
                  }
                }
              }
              frame 30 {
                n196 = Build Array(u16 0 ("element"), u16 0 ("element")) -> (w740:u16[])
                n197 = call-dynamic "Write Multiple Holding Registers.vi"("error in"=w746, "registers to write"=w740, "starting address"=u16 3, "Modbus master in"=w747) -> ("error out"=w744:errorcluster, "Modbus master out"=w745:refnum<class "Modbus Master.lvclass">)  [unwired: 6 in]
              }
              frame 20 {
                n198 = Greater Or Equal?(x=w762, y=u32 5000) -> (x >= y?=w761:bool)
                n199 = case shown="False" w761 {
                  tunnel: ["PLC DONE=0 확인 중" "DONE=0 수신 확인 시간 초과"] -> w760
                  tunnel: [FALSE TRUE] -> w759
                  tunnel: [w773 u16 20] -> w758
                  tunnel: [w774 w777] -> w757
                  tunnel: w756 -> [w774 w781]
                  tunnel: w755 -> [w768 _]
                  frame False {
                    n200 = Equal?(x=w768, y=u16 0) -> (x = y?=w770:bool)
                    n201 = Select(t=u16 30, s=w770, f=u16 20) -> (s? t:f=w773:u16)
                  }
                  frame True {
                    n202 = Bundle By Name(cluster=w781, "status"=TRUE, "code"=5006, "source"="VirtualATE: DONE=0 수신 확인 시간 초과") -> (w777:errorcluster)
                  }
                }
              }
              frame 10 {
                n203 = call-dynamic "Write Single Holding Register.vi"("error in"=w788, "register to write"=u16 0, "address"=u16 5, "Modbus master in"=w791) -> ("error out"=w789:errorcluster, "Modbus master out"=w790:refnum<class "Modbus Master.lvclass">)  [unwired: 6 in]
              }
            }
          }
          frame Default {
            n204 = Equal?(x=w817, y=5002) -> (x = y?=w807:bool)
            n205 = Equal?(x=w817, y=5003) -> (x = y?=w808:bool)
            n206 = Equal?(x=w817, y=5004) -> (x = y?=w809:bool)
            n207 = Equal?(x=w817, y=5005) -> (x = y?=w812:bool)
            n208 = Select(t="검사 요청 철회", s=w812, f="ATE 제어 고장" ("t")) -> (s? t:f=w803:string)
            n209 = Select(t="요청 번호 감소 또는 검사 중 변경", s=w809, f=w803) -> (s? t:f=w802:string)
            n210 = Select(t="PLC 알람 또는 운전 불가", s=w808, f=w802) -> (s? t:f=w801:string)
            n211 = Select(t="PLC 카운터 변경 중단", s=w807, f=w801) -> (s? t:f=w799:string)
            n212 = Bundle By Name(cluster=w819, "status"=TRUE, "code"=w817, "source"=w799) -> (w820:errorcluster)
          }
        }
        n213 = Equal?(x=w113, y=u16 0) -> (x = y?=w124:bool)
        n214 = Equal?(x=w130, y=u16 60) -> (x = y?=w123:bool)
        n215 = And(x=w124, y=w123) -> (x .and. y?=w120:bool)
        n216 = And(x=w119, y=w120) -> (x .and. y?=w118:bool)
        n217 = And(x=w104, y=w118) -> (x .and. y?=w117:bool)
      }
    }
    "PLC_LIVE_OK" <- w49
    "ATE_STATE" <- w33
    "ACTIVE_ID" <- w35
    "ACTIVE_RESULT" <- w34
    "ACTIVE_RECORD" <- w31
    n218 = Unbundle By Name(w53) -> ("status"=w52:bool)
    n219 = Not Equal?(x=w45, y=w33) -> (x != y?=w46:bool)
    n220 = Concatenate Strings("VirtualATE: ", w37) -> (→"처리 메시지":string)
    n221 = Or(x=w52, y="ATE 읽기 정지") -> (x .or. y?=w57:bool)
    n222 = Select(t=w41, s=w46, f=w44) -> (s? t:f=w47:u32)
    n223 = Or(x=w56, y=w57) -> (x .or. y?=w50:bool)
    n224 = Not(x=w50) -> (.not. x?=w51:bool)
    n225 = And(x=w54, y=w51) -> (x .and. y?=→"ATE_READY":bool)
  }
  n226 = call <vilib>:"Clear Errors.vi"("error in (no error)"=w13) -> ("error out"=w12:errorcluster)  [unwired: 5 in, 1 out]
  n227 = case shown="True" w17 {
    tunnel: w16 -> [_ w829]
    tunnel: [w826 w828] -> w15
    tunnel: w12 -> [w826 w827]
    frame False {
    }
    frame True {
      n228 = call-dynamic "Shutdown.vi"("error in"=w827, "Modbus master in"=w829) -> ("error out"=w828:errorcluster)  [unwired: 9 in]
    }
  }
  n229 = Merge Errors(w13, w15) -> (→"error out":errorcluster)
